vi "HTTP Client Abstract Tree.vi"() -> ()   [LabVIEW 2020]
uses:
  Classes/LabVIEW HTTP Client/LabVIEW HTTP Client.lvclass
panel:
  out "Array":string[][](array[string])
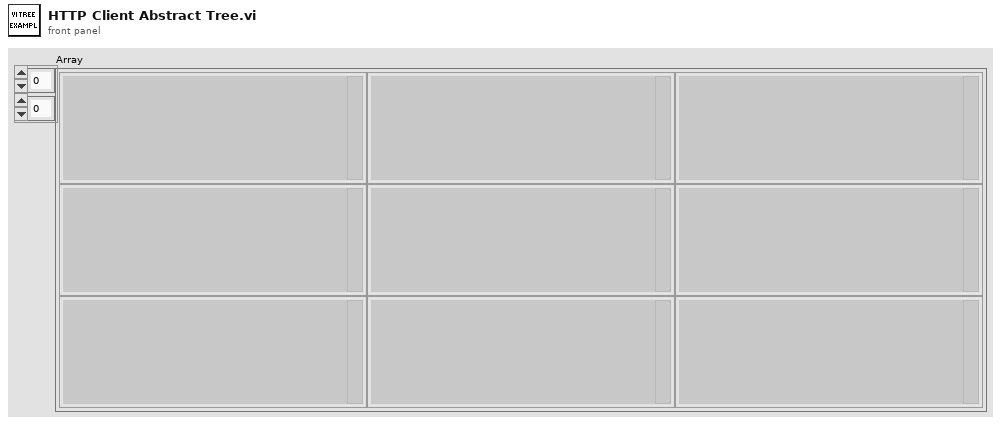
[diagram p1: front panel]
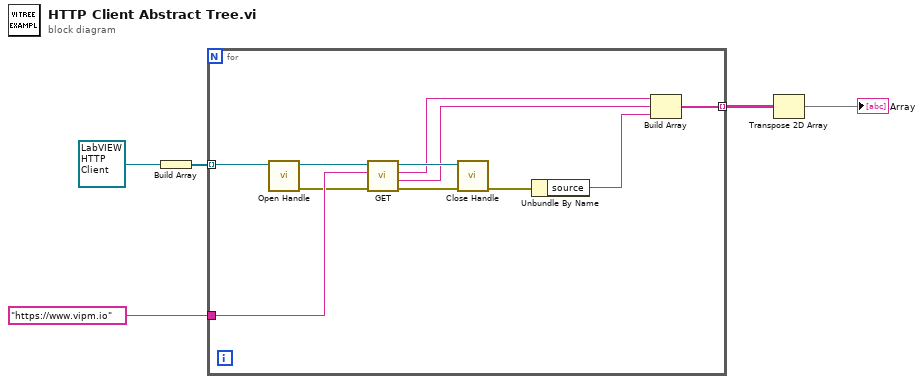
[diagram p0: block diagram]
diagram:
  n1 = Build Array(refnum<class "LabVIEW HTTP Client.lvclass"> refnum ("HTTP Client Base in")) -> (w5:refnum<class "LabVIEW HTTP Client.lvclass">[])
  n2 = for {
    tunnel: w5 -> [w16] mode=indexing
    tunnel: "https://www.vipm.io" ("url") -> [w13]
    tunnel: [w7] -> w3 mode=indexing
    n3 = call-dynamic "Open Handle.vi"("HTTP Client Base in"=w16) -> ("error out"=w12:errorcluster, "HTTP Client Base out"=w15:refnum<class "LabVIEW HTTP Client.lvclass">)  [unwired: 9 in]
    n4 = call-dynamic "GET.vi"("error in (no error)"=w12, "url"=w13, "HTTP Client Base in"=w15) -> ("error out"=w11:errorcluster, "body"=w6:string, "headers"=w9:string, "HTTP Client Base out"=w14:refnum<class "LabVIEW HTTP Client.lvclass">)  [unwired: 4 in, 1 out]
    n5 = call-dynamic "Close Handle.vi"("error in (no error)"=w11, "HTTP Client Base in"=w14) -> ("error out"=w10:errorcluster)  [unwired: 8 in, 1 out]
    n6 = Unbundle By Name(w10) -> ("source"=w8:string)
    n7 = Build Array(w9, w6, w8) -> (w7:string[])
  }
  n8 = Transpose 2D Array(2D array=w3) -> (transposed array=→"Array":string[][])
